vi "Read Program List.vi"() -> (3 "Program List":string[](array[string]))   [LabVIEW 2025]
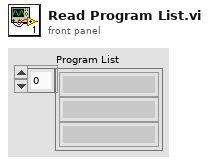
[diagram p1: front panel]
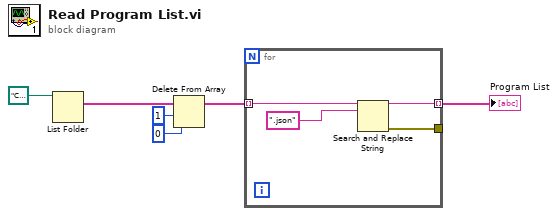
[diagram p0: block diagram]
diagram:
  n1 = List Folder(path=path "C:/Users/Public/Documents/torque-test-station/programs") -> (filenames=w5:string[])  [unwired: 3 in, 3 out]
  n2 = Delete From Array(array=w5, length=1, index=0) -> (array with subset deleted=w2:string[])  [unwired: 1 out]
  n3 = for {
    tunnel: w2 -> [w10] mode=indexing
    tunnel: [w8] -> _
    tunnel: [w7] -> w1 mode=indexing
    n4 = Search and Replace String(input string=w10, search string=".json") -> (result string=w7:string, error out=w8:errorcluster)  [unwired: 6 in, 2 out]
  }
  "Program List" <- w1
